vi "Global.vi"() -> ()   [LabVIEW 2017]
panel:
  in  "Chat":string
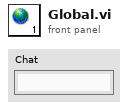
[diagram p1: front panel]
diagram:
